vi "Vides extra.vi"(4 "y depredador":dbl, 6 "x depredador":dbl, 7 "Vides inicials":i32, 9 "y aleatoria":dbl, 10 "x aleatoria":dbl, 11 "Boolean":bool) -> (2 "vides finals":i32, 3 "Cluster":cluster{dbl[], dbl[]})   [LabVIEW 2023]
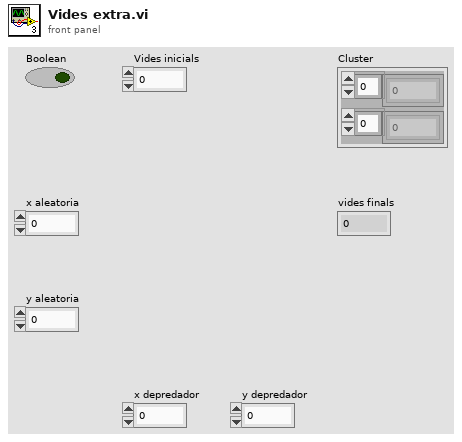
[diagram p1: front panel]
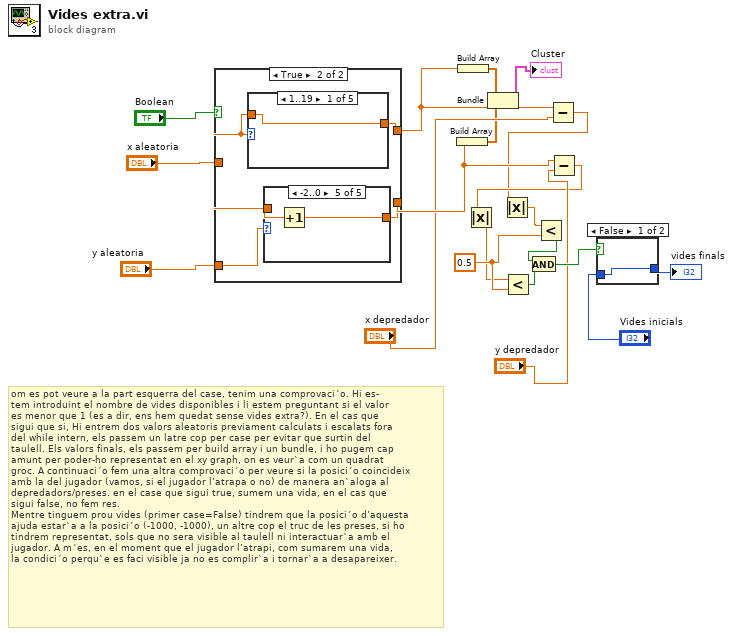
[diagram p0: block diagram]
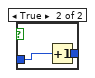
[diagram p2: hidden frame]
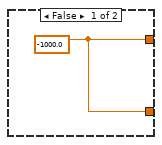
[diagram p3: hidden frame]
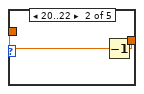
[diagram p5: hidden frame]
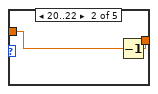
[diagram p8: hidden frame]
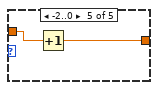
[diagram p11: hidden frame]
diagram:
  w16 = 0.5
  # "om es pot veure a la part esquerra del case, tenim una comprovaci´o. Hi es-\ntem introduint el nombre de vides disponibles i li estem preguntant si el valor\nes menor que 1 (es a dir, ens hem quedat sense vides extra?). En el cas que\nsigui que si, Hi entrem dos valors aleatoris previament calculats i escalats fora\ndel while intern, els passem un latre cop per case per evitar que surtin del\ntaulell. Els valors finals, els passem per build array i un bundle, i ho pugem cap\namunt per poder-ho representat en el xy graph, on es veur`a com un quadrat\ngroc. A continuaci´o fem una altra comprovaci´o per veure si la posici´o coincideix\namb la del jugador (vamos, si el jugador l’atrapa o no) de manera an`aloga al\ndepredadors/preses. en el case que sigui true, sumem una vida, en el cas que\nsigui false, no fem res.\nMentre tinguem prou vides (primer case=False) tindrem que la posici´o d’aquesta\najuda estar`a a la posici´o (-1000, -1000), un altre cop el truc de les preses, si ho\ntindrem representat, sols que no sera visible al taulell ni interactuar`a amb el\njugador. A m´es, en el moment que el jugador l’atrapi, com sumarem una vida,\nla condici´o perqu`e es faci visible ja no es complir`a i tornar`a a desapareixer."
  n1 = case shown="True" "Boolean" {
    tunnel: [w21 w25] -> w17
    tunnel: [w21 w24] -> w11
    tunnel: "y aleatoria" -> [_ w23]
    tunnel: "x aleatoria" -> [_ w22]
    frame False {
      w21 = -1000.0
    }
    frame True {
      n2 = case shown="1..19" w22 {
        tunnel: [w33 w35 w36 w37 w39] -> w25
        tunnel: w22 -> [w33 w34 w36 w37 w38]
        frame 1..19 {
        }
        frame 20..22 {
          n3 = Decrement(x=w34) -> (x-1=w35:dbl)
        }
        frame 23.. {
        }
        frame ..-3 {
        }
        frame -2..0 {
          n4 = Increment(x=w38) -> (x+1=w39:dbl)
        }
      }
      n5 = case shown="-2..0" w23 {
        tunnel: [w26 w28 w29 w30 w32] -> w24
        tunnel: w23 -> [w26 w27 w29 w30 w31]
        frame 1..19 {
        }
        frame 20..22 {
          n6 = Decrement(x=w27) -> (x-1=w28:dbl)
        }
        frame 23.. {
        }
        frame ..-3 {
        }
        frame -2..0 {
          n7 = Increment(x=w31) -> (x+1=w32:dbl)
        }
      }
    }
  }
  n8 = Build Array(w11) -> (w3:dbl[])
  n9 = Build Array(w17) -> (w2:dbl[])
  n10 = Bundle(w2, w3) -> (→"Cluster":cluster{dbl[], dbl[]})  [unwired: 1 in]
  n11 = Subtract(x=w17, y="x depredador") -> (x-y=w6:dbl)
  n12 = Absolute Value(x=w6) -> (abs(x)=w7:dbl)
  n13 = Less?(x=w7, y=w16) -> (x < y?=w4:bool)
  n14 = Subtract(x=w11, y="y depredador") -> (x-y=w8:dbl)
  n15 = Absolute Value(x=w8) -> (abs(x)=w9:dbl)
  n16 = Less?(x=w9, y=w16) -> (x < y?=w5:bool)
  n17 = And(x=w4, y=w5) -> (x .and. y?=w14:bool)
  n18 = case shown="False" w14 {
    tunnel: "Vides inicials" -> [w40 w42]
    tunnel: [w40 w41] -> w15
    frame False {
    }
    frame True {
      n19 = Increment(x=w42) -> (x+1=w41:i32)
    }
  }
  "vides finals" <- w15
